vi "CfgManager.Text Test Launcher.vi"() -> ()   [LabVIEW 2013]
uses:
  source/Manager.Text/ConfigManager.Text.lvclass
  source/Manager/Decompose KVPs.vi
  source/Manager/Write.vi
  source/Manager/ConfigManager.lvclass
panel:
  out "array of clusters":variant
  out "Keys":string[](array[string])
  out "modified configuration":variant
  out "error out":errorcluster
  out "initial configuration":variant
  out "filepath":path
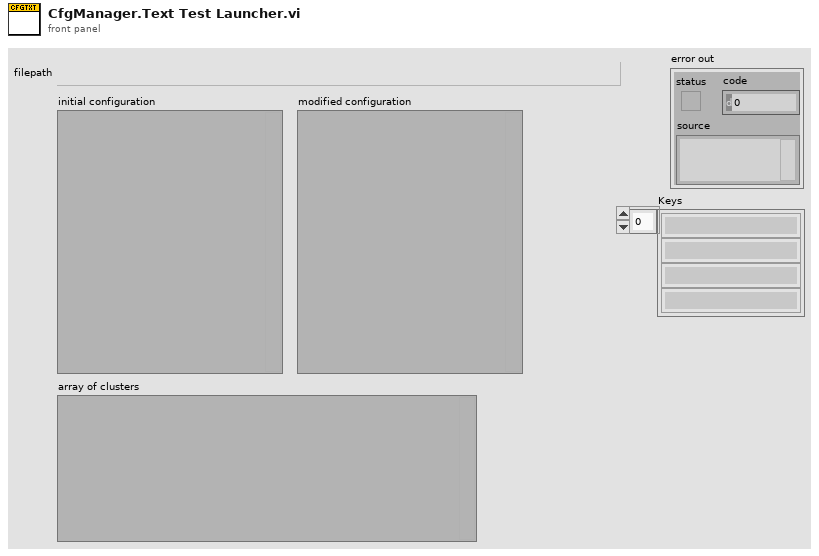
[diagram p1: front panel]
types:
  T1 = cluster{"String":string, "Numeric":dbl, "Boolean":bool, "array":dbl[]}
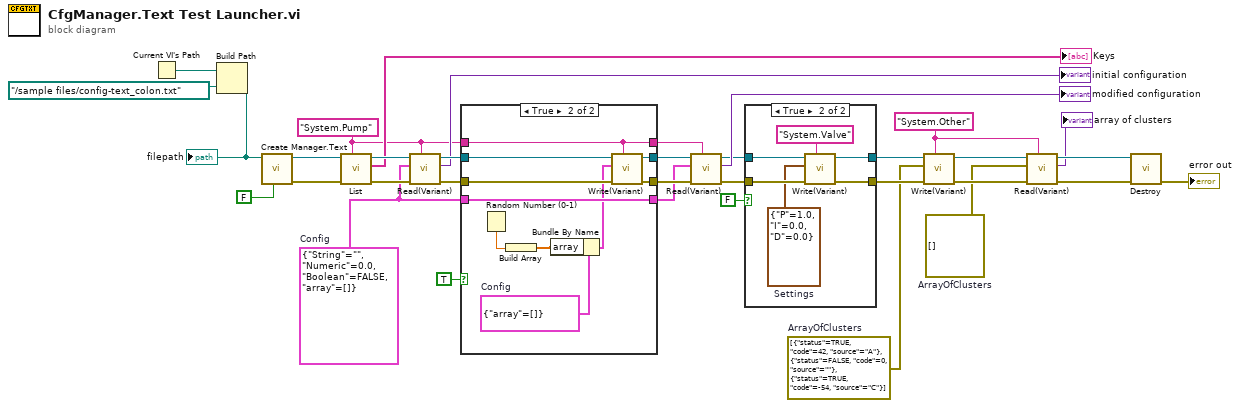
[diagram p0: block diagram]
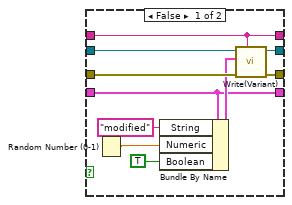
[diagram p2: hidden frame]
diagram:
  w2 = errorcluster[] []  # ArrayOfClusters
  w4 = "System.Other" ("Qualified Name")
  w3 = errorcluster[] [{"status"=TRUE, "code"=42, "source"="A"}, {"status"=FALSE, "code"=0, "source"=""}, {"status"=TRUE, "code"=-54, "source"="C"}]  # ArrayOfClusters
  w19 = "System.Pump" ("Qualified Name")
  w16 = T1 {"String"="", "Numeric"=0.0, "Boolean"=FALSE, "array"=[]}  # Config
  n1 = Current VI's Path() -> (path=w13:path)
  n2 = Build Path(base path=w13, name or relative path=path "../sample files/config-text_colon.txt" ("filepath 2")) -> (appended path=w11:path)
  "filepath" <- w11
  n3 = call "Create Manager.Text.vi"("read-only?"=FALSE, "filepath"=w11) -> ("error out"=w27:errorcluster, "ConfigManager.Text out"=w28:refnum<class "ConfigManager.Text.lvclass">)  [unwired: 7 in, 1 out]
  n4 = call "List.vi"("Qualified Name"=w19, "error in (no error)"=w27, "ConfigManager in"=w28) -> ("error out"=w26:errorcluster, "Keys"=→"Keys":string[], "ConfigManager out"=w25:refnum<class "ConfigManager.Text.lvclass">)  [unwired: 6 in]
  n5 = call "Read(Variant).vi"("Qualified Name"=w19, "error in (no error)"=w26, "Type"=w16, "ConfigManager in"=w25) -> ("error out"=w32:errorcluster, "value"=→"initial configuration":variant, "ConfigManager out"=w33:refnum<class "ConfigManager.Text.lvclass">)  [unwired: 3 in, 2 out]
  n6 = case shown="True" TRUE {
    tunnel: w33 -> [w41 w54]
    tunnel: w32 -> [w40 w53]
    tunnel: [w43 w52] -> w31
    tunnel: [w42 w51] -> w30
    tunnel: w19 -> [w44 w50]
    tunnel: [w44 w50] -> w17
    tunnel: w16 -> [w35 w49]
    tunnel: [w35 w49] -> w15
    frame False {
      n7 = Random Number (0-1)() -> (number: 0 to 1=w37:dbl)
      n8 = Bundle By Name(cluster=w35, "String"="modified", "Numeric"=w37, "Boolean"=TRUE) -> (w36:T1)
      n9 = call "Write(Variant).vi"("Qualified Name"=w44, "error in (no error)"=w40, "value"=w36, "ConfigManager in"=w41) -> ("error out"=w42:errorcluster, "ConfigManager out"=w43:refnum<class "ConfigManager.Text.lvclass">)  [unwired: 5 in, 1 out]
    }
    frame True {
      w48 = cluster{"array":dbl[]} {"array"=[]}  # Config
      n10 = Random Number (0-1)() -> (number: 0 to 1=w46:dbl)
      n11 = Build Array(w46) -> (w45:dbl[])
      n12 = Bundle By Name(cluster=w48, "array"=w45) -> (w47:cluster{"array":dbl[]})
      n13 = call "Write(Variant).vi"("Qualified Name"=w50, "error in (no error)"=w53, "value"=w47, "ConfigManager in"=w54) -> ("error out"=w51:errorcluster, "ConfigManager out"=w52:refnum<class "ConfigManager.Text.lvclass">)  [unwired: 5 in, 1 out]
    }
  }
  n14 = call "Read(Variant).vi"("Qualified Name"=w17, "error in (no error)"=w30, "Type"=w15, "ConfigManager in"=w31) -> ("error out"=w21:errorcluster, "value"=→"modified configuration":variant, "ConfigManager out"=w22:refnum<class "ConfigManager.Text.lvclass">)  [unwired: 3 in, 2 out]
  n15 = case shown="True" FALSE {
    tunnel: w22 -> [w56 w62]
    tunnel: [w56 w61] -> w10
    tunnel: w21 -> [w55 w60]
    tunnel: [w55 w59] -> w6
    frame False {
    }
    frame True {
      w57 = cluster{"P":dbl, "I":dbl, "D":dbl} {"P"=1.0, "I"=0.0, "D"=0.0}  # Settings
      n16 = call "Write(Variant).vi"("Qualified Name"="System.Valve", "error in (no error)"=w60, "value"=w57, "ConfigManager in"=w62) -> ("error out"=w59:errorcluster, "ConfigManager out"=w61:refnum<class "ConfigManager.Text.lvclass">)  [unwired: 5 in, 1 out]
    }
  }
  n17 = call "Write(Variant).vi"("Qualified Name"=w4, "error in (no error)"=w6, "value"=w3, "ConfigManager in"=w10) -> ("error out"=w7:errorcluster, "ConfigManager out"=w9:refnum<class "ConfigManager.Text.lvclass">)  [unwired: 5 in, 1 out]
  n18 = call "Read(Variant).vi"("Qualified Name"=w4, "error in (no error)"=w7, "Type"=w2, "ConfigManager in"=w9) -> ("error out"=w5:errorcluster, "value"=→"array of clusters":variant, "ConfigManager out"=w8:refnum<class "ConfigManager.Text.lvclass">)  [unwired: 3 in, 2 out]
  n19 = call-dynamic "Destroy.vi"("error in (no error)"=w5, "ConfigManager.Text in"=w8) -> ("error out"=→"error out":errorcluster)  [unwired: 8 in, 1 out]
